vi "FuncVI-Alias.vi"(5 "InstanceRef":T2, 9 "arg list":T1[](array[typedef]) {"num" format="%.2f"}) -> (0 "error out":bool, 3 "result":T1 {"num" format="%.2f"})   [LabVIEW 2021]
doc: "::: CalcExpress Toolkit :::\nCopyright (c) 2000-2026 Konstantin Shifershteyn. All rights reserved."
uses:
  cetypes.llb/CalcExpress Function Argument Info.ctl
  cetypes.llb/CalcExpress Instance RefNum.ctl
panel:
  in  "max arg num":i32=3
  in  "min arg num":i32=2
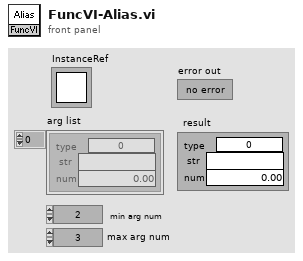
[diagram p1: front panel]
types:
  T1 = typedef "CalcExpress Function Argument Info.ctl" = cluster{"type":u32, "str":string, "num":dbl}
  T2 = typedef "CalcExpress Instance RefNum.ctl" = refnum<k1>
  T3 = enum32{"String", "DBL Number", "identifier", "1D Array of DBL", "2D Array of DBL", "CDB Number", "1D Array of CDB", "2D Array of CDB", "1D Array of String", "2D Array of String", "Unknown data type"}
  T4 = cluster{"index":i32, "data type":enum32{"String", "DBL Number", "identifier", "1D Array of DBL", "2D Array of DBL", "CDB Number", "1D Array of CDB", "2D Array of CDB", "1D Array of String", "2D Array of String", "Unknown data type"}, "default num":dbl, "default str":string}[]
  T5 = typedef "VarMan Variable Context Handle.ctl" = i32
  T6 = cluster{"data type":enum32{"String", "DBL Number", "identifier", "1D Array of DBL", "2D Array of DBL", "CDB Number", "1D Array of CDB", "2D Array of CDB", "1D Array of String", "2D Array of String", "Unknown data type"}, string, dbl}
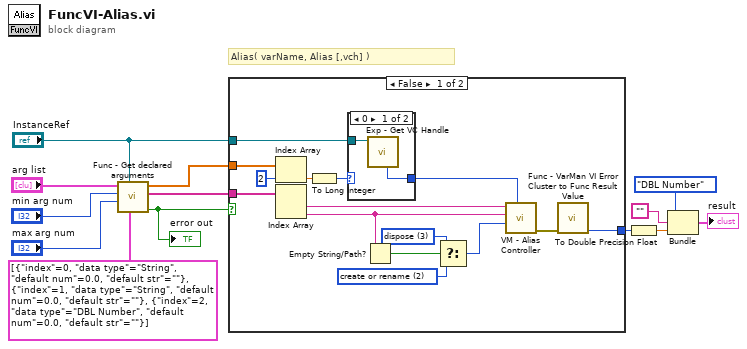
[diagram p0: block diagram]
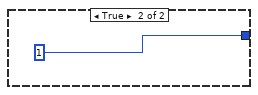
[diagram p3: hidden frame]
diagram:
  # "Alias( varName, Alias [,vch] )"
  n1 = call "Func - Get declared arguments.vi"("arg descriptors"=T4 [{"index"=0, "data type"=enum."String", "default num"=0.0, "default str"=""}, {"index"=1, "data type"=enum."String", "default num"=0.0, "default str"=""}, {"index"=2, "data type"=enum."DBL Number", "default num"=0.0, "default str"=""}], "InstanceRef"="InstanceRef", "max arg num"="max arg num", "min arg num"="min arg num", "arg list"="arg list") -> ("error out"=w12:bool, "str list"=w8:string[], "num list"=w1:dbl[])  [unwired: 3 in, 1 out]
  "error out" <- w12
  n2 = case shown="False" w12 {
    tunnel: w1 -> [w24 _]
    tunnel: w8 -> [w22 _]
    tunnel: [w15 1 ("code")] -> w7
    tunnel: "InstanceRef" -> [w28 _]
    frame False {
      w18 = u32 3 items=["nop", "create", "create or rename", "dispose"] ("action")
      w19 = u32 2 items=["nop", "create", "create or rename", "dispose"] ("action")
      n3 = Index Array(array=w24, index=2) -> (element=w26:dbl)
      n4 = Index Array(array=w22) -> (element #1=w21:string, element #2=w14:string)  [unwired: 2 in]
      n5 = To Long Integer(number=w26) -> (32bit integer=w23:i32)
      n6 = case shown="0" w23 {
        selector: w23 -> [_ w31]
        tunnel: w28 -> [w30 _]
        tunnel: [w29 w31] -> w27
        frame 0 {
          n7 = call "Exp - Get VC Handle.vi"("InstanceRef"=w30) -> ("VC Handle"=w29:T5)  [unwired: 5 in, 3 out]
        }
        frame 1, Default {
        }
      }
      n8 = Empty String/Path?(string/path=w14) -> (empty?=w20:bool)
      n9 = Select(t=w18, s=w20, f=w19) -> (s? t:f=w17:u32)
      n10 = call "VM - Alias Controller.vi"("VC Handle"=w27, "action"=w17, "alias"=w14, "name_spec"=w21) -> ("error out"=w16:errorcluster)  [unwired: 4 in, 3 out]
      n11 = call "Func - VarMan VI Error Cluster to Func Result Value.vi"("VarMan VI error in"=w16) -> ("CE Function Result Value"=w15:i32)  [unwired: 10 in]
    }
    frame True {
    }
  }
  n12 = To Double Precision Float(number=w7) -> (double precision float=w6:dbl)
  n13 = Bundle("data type"=T3."DBL Number", "", w6) -> (→"result":T6)  [unwired: 1 in]
